vi "Report.vi"(8 "error in":errorcluster, 11 "file in":path) -> (0 "error out":errorcluster={"status"=TRUE, "code"=118, "source"="TDMS Open in TDMS - File Viewer with Flat Layout.vi"}, 3 "file out":path)   [LabVIEW 2020]
uses:
  <vilib>/Utility/TDMS File Viewer/NI_TDMS File Viewer.lvlib
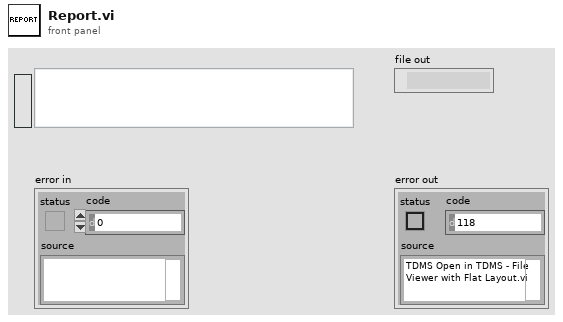
[diagram p1: front panel]
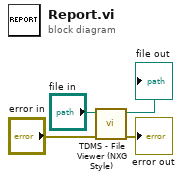
[diagram p0: block diagram]
diagram:
  n1 = call <vilib>:"TDMS - File Viewer (NXG Style).vi"("error in"="error in", "file in"="file in") -> ("error out"=→"error out":errorcluster, "file out"=→"file out":path)  [unwired: 8 in]
